vi "Test REV reservation.vi"() -> ()   [LabVIEW 2026]
uses:
  <vilib>/REV Custom Controls/REVSparkRefnum.ctl
  <vilib>/REV Custom Controls/Spark Output Control Type.ctl
  <vilib>/REVLibDriver/REVLibDriver.lvlib
panel:
  in  "Setpoint 2":dbl(slide) scale=-1.0..1.0
  in  "Setpoint":dbl(slide) scale=-1.0..1.0
  out "error out 4":errorcluster
  out "Spark refnum 2":T1
  out "Spark refnum":T1
  out "error out 3":errorcluster
  out "error out 2":errorcluster
  out "error out":errorcluster
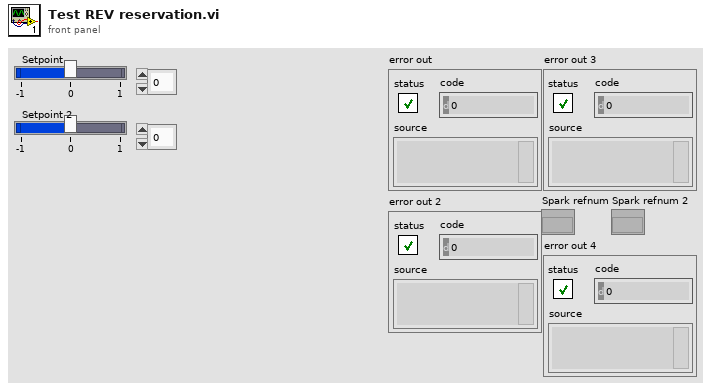
[diagram p1: front panel]
types:
  T1 = typedef "REVLibDriver.lvlib/REVSparkRefnum.ctl" = refnum<k20>
  T2 = typedef "REVLibDriver.lvlib/Spark Output Control Type.ctl" = enum16{"Percent VBus", "Velocity", "Voltage", "Position", "Current", "MAXMotion Position", "MAXMotion Velocity"}
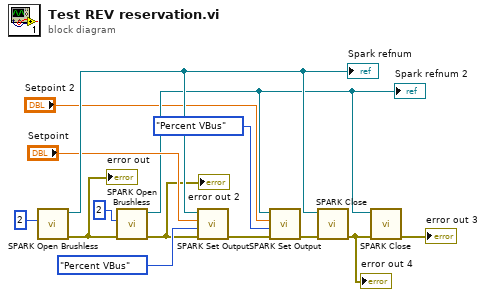
[diagram p0: block diagram]
diagram:
  n1 = call <vilib>:"SPARK Open Brushless.vi"("deviceId"=2) -> ("error out"=w13:errorcluster, "Spark refnum"=w10:T1)  [unwired: 9 in]
  "error out" <- w13
  "Spark refnum" <- w10
  n2 = call <vilib>:"SPARK Open Brushless.vi"("error in"=w13, "deviceId"=2) -> ("error out"=w1:errorcluster, "Spark refnum"=w5:T1)  [unwired: 8 in]
  "error out 2" <- w1
  "Spark refnum 2" <- w5
  n3 = call <vilib>:"SPARK Set Output.vi"("error in (no error)"=w1, "Control Mode"=Spark_Output_Control_Type."Percent VBus", "Setpoint"="Setpoint", "Spark refnum"=w10) -> ("error out"=w7:errorcluster)  [unwired: 6 in, 1 out]
  n4 = call <vilib>:"SPARK Set Output.vi"("error in (no error)"=w7, "Control Mode"=Spark_Output_Control_Type."Percent VBus", "Setpoint"="Setpoint 2", "Spark refnum"=w5) -> ("error out"=w3:errorcluster)  [unwired: 6 in, 1 out]
  n5 = call <vilib>:"SPARK Close.vi"("error in (no error)"=w3, "Spark refnum"=w10) -> ("error out"=w2:errorcluster)  [unwired: 9 in]
  "error out 4" <- w2
  n6 = call <vilib>:"SPARK Close.vi"("error in (no error)"=w2, "Spark refnum"=w5) -> ("error out"=→"error out 3":errorcluster)  [unwired: 9 in]
